vi "Initialize Generate with Scheduler.vi"(8 "error in (no error)":errorcluster, 10 "PCL (usec)":u32, 11 "OnCompile Variables":T1={"Name"="", "XNET Settings"={"Database"="", "Cluster"="", "Port"="", "Baud rate [Bd]"=500000, "Termination"=1, "CAN I/O Mode"=0, "FD Baud rate [Bd]"=500000, "Priority"=100, "Use Legacy"=FALSE, "FD ISO Mode"=0, "Default Max Counter Value"=0.0, "Default Protect Type"=enum."Arb ID + Bytes Checksum with Inversion", "Include All Channels"=FALSE}, "Frames"=[], "986x Support"={"Enable"=FALSE, "RIO Device"="", "Bitfile"=path ""}, "Incoming Frames"=[]} {"Incoming Frames"."Protection Configurations"."CRC Channels"."Data Type" items=["Signed", "Unsigned", "IEEE Float"]; "XNET Settings"."FD ISO Mode" items=["ISO", "Non ISO", "ISO Legacy"]; "XNET Settings"."CAN I/O Mode" items=["CAN 2.0", "CAN FD", "CAN FD+BRS"]; "XNET Settings"."Termination" items=["Off", "On"]; "Frames"."Protection Configurations"."CRC Channels"."Data Type" items=["Signed", "Unsigned", "IEEE Float"]}) -> (0 "error out":errorcluster, 2 "RT Configuration":T11={"Name"="", "Priority"=100, "XNET Settings"={"Database"="", "Cluster"="", "Port"="", "Baud rate [Bd]"=0, "Termination"=0, "CAN I/O Mode"=0, "FD Baud rate [Bd]"=500000, "Priority"=100, "Use Legacy"=FALSE, "FD ISO Mode"=0, "Default Max Counter Value"=0.0, "Default Protect Type"=enum."Arb ID + Bytes Checksum with Inversion", "Include All Channels"=FALSE}, "FPGA Session"=0, "Outgoing CAN Session"="", "Outgoing Cyclic Frame Count"=0, "Outgoing Cyclic Frames"=[], "Outgoing Event Frame Count"=0, "Outgoing Event Frames"=[], "Incoming CAN Session"="", "Incoming Frame Count"=0, "Incoming Frames"=[], "Incoming Values"={"Signal Values"=[], "Signal Invalid Values"=[], "ProtCtr Sig Values"=[], "Timestamps"=[], "Time Differences"=[], "IDs"=[]}} {"Outgoing Event Frames"."Protection Configurations"."CRC Channels"."Data Type" items=["Signed", "Unsigned", "IEEE Float"]; "Incoming Frames"."Protection Configurations"."CRC Channels"."Data Type" items=["Signed", "Unsigned", "IEEE Float"]; "XNET Settings"."FD ISO Mode" items=["ISO", "Non ISO", "ISO Legacy"]; "XNET Settings"."CAN I/O Mode" items=["CAN 2.0", "CAN FD", "CAN FD+BRS"]; "XNET Settings"."Termination" items=["Off", "On"]; "Outgoing Cyclic Frames"."Protection Configurations"."CRC Channels"."Data Type" items=["Signed", "Unsigned", "IEEE Float"]}, 3 "OnCompile Variables out":T1={"Name"="", "XNET Settings"={"Database"="", "Cluster"="", "Port"="", "Baud rate [Bd]"=500000, "Termination"=1, "CAN I/O Mode"=0, "FD Baud rate [Bd]"=500000, "Priority"=100, "Use Legacy"=FALSE, "FD ISO Mode"=0, "Default Max Counter Value"=0.0, "Default Protect Type"=enum."Arb ID + Bytes Checksum with Inversion", "Include All Channels"=FALSE}, "Frames"=[], "986x Support"={"Enable"=FALSE, "RIO Device"="", "Bitfile"=path ""}, "Incoming Frames"=[]} {"Incoming Frames"."Protection Configurations"."CRC Channels"."Data Type" items=["Signed", "Unsigned", "IEEE Float"]; "XNET Settings"."FD ISO Mode" items=["ISO", "Non ISO", "ISO Legacy"]; "XNET Settings"."CAN I/O Mode" items=["CAN 2.0", "CAN FD", "CAN FD+BRS"]; "XNET Settings"."Termination" items=["Off", "On"]; "Frames"."Protection Configurations"."CRC Channels"."Data Type" items=["Signed", "Unsigned", "IEEE Float"]})   [LabVIEW 2026]
uses:
  Addon Shared/Types/Exported.OnCompile.ctl
  Addon Shared/Types/XNET Settings.ctl
  SubModules/Frame-Protection-Support/Source/Shared/Types/Protection Type.ctl
  SubModules/Frame-Protection-Support/Source/Shared/Types/Exported Frame Settings.ctl
  SubModules/Frame-Protection-Support/Source/Shared/Types/Exported Frame Type.ctl
  SubModules/Frame-Protection-Support/Source/Shared/Types/Exported Protection Settings.ctl
  SubModules/Frame-Protection-Support/Source/Shared/Types/XNET Signal Configuration.ctl
  SubModules/Frame-Protection-Support/Source/Shared/Types/Exported Counter Settings.ctl
  SubModules/Frame-Protection-Support/Source/Shared/Types/Exported Event Trigger Type.ctl
  Addon Shared/Types/986x.ctl
  Types/RT Async Engine Settings.ctl
  SubModules/Frame-Protection-Support/Source/Engine/Types/RT Frame Settings.ctl
  SubModules/Frame-Protection-Support/Source/Engine/Types/RT Protection Configuration.ctl
  SubModules/Frame-Protection-Support/Source/Engine/Types/RT Frame Incoming Values.ctl
  Bitfile.Download.vi
  <vilib>/Utility/libraryn.llb/Check if File or Folder Exists.vi
  <vilib>/Utility/error.llb/Error Cluster From Error Code.vi
  <vilib>/rvi/Utilities/XML/nirviXML_GetValue.vi
  <vilib>/rvi/Utilities/XML/nirviXML_GetValue_String.vi
  <vilib>/xnet/xnet.llb/XNET Create Session (Frame Output Stream).vi
  <vilib>/xnet/xnet.llb/XNET Create Session (Conversion).vi
  SubModules/Frame-Protection-Support/Source/Shared/Protection and Counter Support Shared.lvlib
  SubModules/Frame-Protection-Support/Source/Engine/Protection and Counter Support Engine.lvlib
  Protection and Counter Addon Engine.lvlib
  <resource>/objmgr/xnet.rc
  Addon Shared/Protection and Counter Addon Shared.lvlib
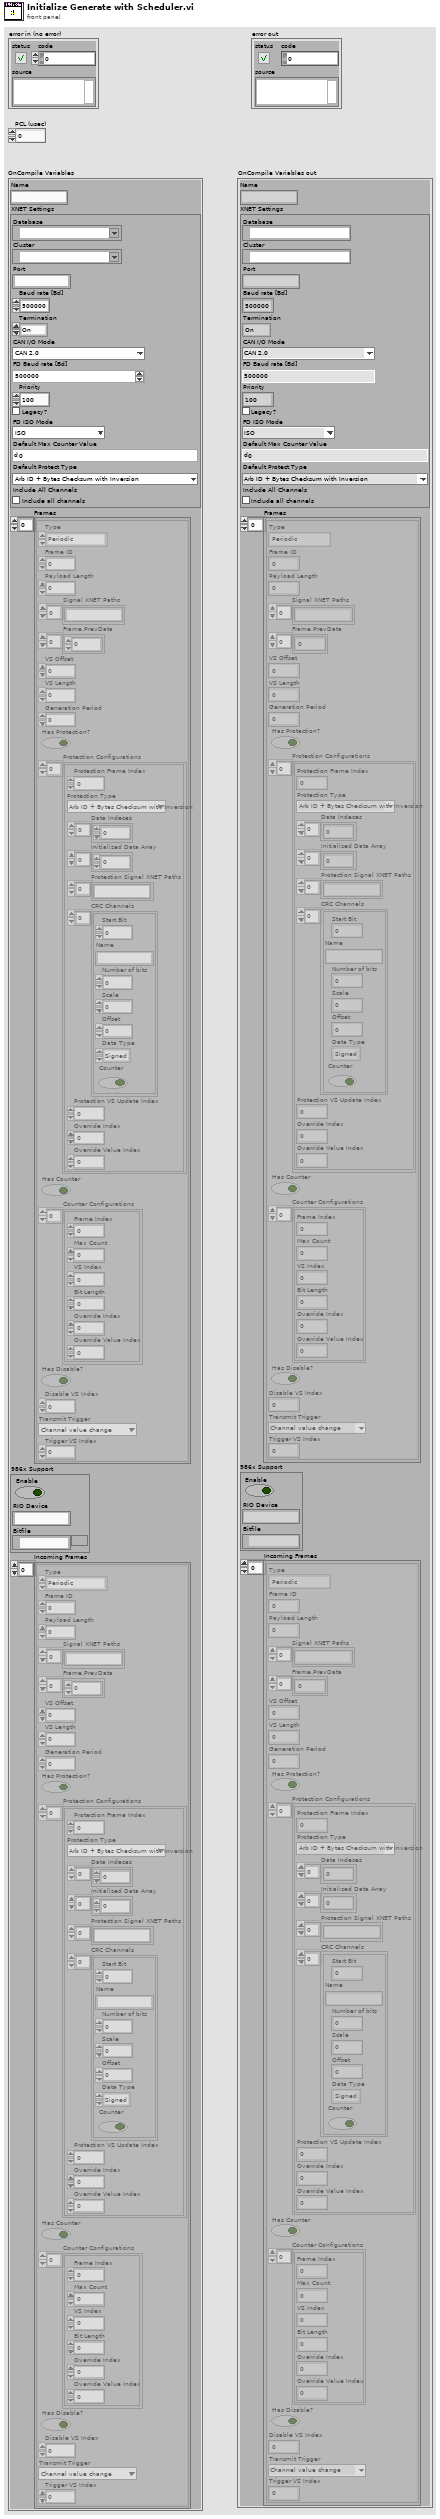
[diagram p1: front panel]
types:
  T1 = typedef "Protection and Counter Addon Shared.lvlib/Exported.OnCompile.ctl" = cluster{"Name":string, "XNET Settings":T2, "Frames":T4[], "986x Support":T10, "Incoming Frames":T4[]}
  T2 = typedef "Protection and Counter Addon Shared.lvlib/XNET Settings.ctl" = cluster{"Database":refnum<k21>, "Cluster":refnum<k21>, "Port":string, "Baud rate [Bd]":u64, "Termination":u32, "CAN I/O Mode":u32, "FD Baud rate [Bd]":u64, "Priority":i32, "Use Legacy":bool, "FD ISO Mode":u32, "Default Max Counter Value":dbl, "Default Protect Type":T3, "Include All Channels":bool}
  T3 = typedef "Protection and Counter Support Shared.lvlib/Protection Type.ctl" = enum16{"Arb ID + Bytes Checksum with Inversion", "Arb ID + Bytes CRC with Inversion", "Reversed Raw Signal Checksum with Inversion", "Concatenated Two's Compliment"}
  T4 = typedef "Protection and Counter Support Shared.lvlib/Exported Frame Settings.ctl" = cluster{"Type":T5, "Frame ID":u32, "Payload Length":u32, "Signal XNET Paths":string[], "Frame.PrevData":dbl[], "VS Offset":i32, "VS Length":i32, "Generation Period":u32, "Has Protection?":bool, "Protection Configurations":T6[], "Has Counter":bool, "Counter Configurations":T8[], "Has Disable?":bool, "Disable VS Index":i32, "Transmit Trigger":T9, "Trigger VS Index":i32}
  T5 = typedef "Protection and Counter Support Shared.lvlib/Exported Frame Type.ctl" = enum16{"Periodic", "Event", "Periodic/Event"}
  T6 = typedef "Protection and Counter Support Shared.lvlib/Exported Protection Settings.ctl" = cluster{"Protection Frame Index":i32, "Protection Type":T3, "Data Indeces":i32[], "Initialized Data Array":dbl[], "Protection Signal XNET Paths":string[], "CRC Channels":T7[], "Protection VS Update Index":i32, "Override Index":i32, "Override Value Index":i32}
  T7 = typedef "Protection and Counter Support Shared.lvlib/XNET Signal Configuration.ctl" = cluster{"Start Bit":i32, "Name":string, "Number of bits":i32, "Scale":dbl, "Offset":dbl, "Data Type":u32, "Counter":bool}
  T8 = typedef "Protection and Counter Support Shared.lvlib/Exported Counter Settings.ctl" = cluster{"Frame Index":i32, "Max Count":dbl, "VS Index":i32, "Bit Length":i64, "Override Index":i32, "Override Value Index":i32}
  T9 = typedef "Protection and Counter Support Shared.lvlib/Exported Event Trigger Type.ctl" = enum16{"Channel value change", "Trigger channel (not zero)", "Channel value change or trigger channel (not zero)", "Trigger channel (any value change)", "Channel value change or trigger channel (any value change)"}
  T10 = typedef "Protection and Counter Addon Shared.lvlib/986x.ctl" = cluster{"Enable":bool, "RIO Device":string, "Bitfile":path}
  T11 = typedef "Protection and Counter Addon Engine.lvlib/RT Async Engine Settings.ctl" = cluster{"Name":string, "Priority":i32, "XNET Settings":T2, "FPGA Session":u32, "Outgoing CAN Session":refnum<k21>, "Outgoing Cyclic Frame Count":i32, "Outgoing Cyclic Frames":T12[], "Outgoing Event Frame Count":i32, "Outgoing Event Frames":T12[], "Incoming CAN Session":refnum<k21>, "Incoming Frame Count":i32, "Incoming Frames":T12[], "Incoming Values":T14}
  T12 = typedef "Protection and Counter Support Engine.lvlib/RT Frame Settings.ctl" = cluster{"Type":T5, "Frame ID":u32, "Payload Length":u32, "VS Offset":i32, "VS Length":i32, "Frame Conversion":refnum<k21>, "Frame.Data":dbl[], "Generation Period":u32, "Time Since Last Generation":u32, "Generation Iterations":u32, "Generation Counter":u32, "Has Protection?":bool, "Protection Configurations":T13[], "Has Counter?":bool, "Counter Configurations":T8[], "Has Disable?":bool, "Disable VS Index":i32, "Transmit Trigger":T9, "Trigger VS Index":i32}
  T13 = typedef "Protection and Counter Support Engine.lvlib/RT Protection Configuration.ctl" = cluster{"Protection Frame Index":i32, "Protection Type":T3, "Data Indeces":i32[], "Data Array":dbl[], "Check Sum Conversion":refnum<k21>, "CRC Channels":T7[], "Protection VS Index":i32, "Counter Data Index":i32, "Override Index":i32, "Override Value Index":i32}
  T14 = typedef "Protection and Counter Support Engine.lvlib/RT Frame Incoming Values.ctl" = cluster{"Signal Values":dbl[], "Signal Invalid Values":dbl[], "ProtCtr Sig Values":dbl[], "Timestamps":timestamp[], "Time Differences":dbl[], "IDs":u32[]}
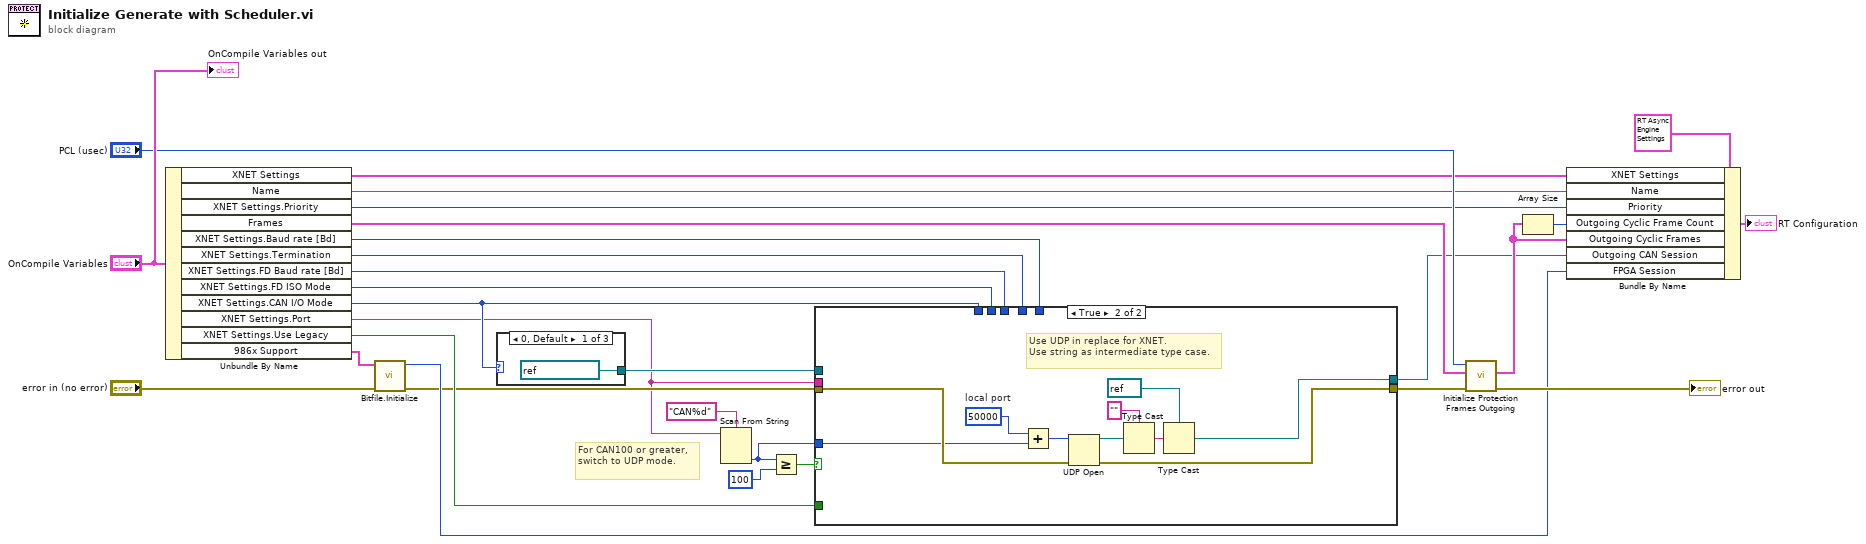
[diagram p0: block diagram]
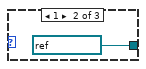
[diagram p2: hidden frame]
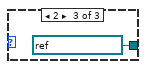
[diagram p3: hidden frame]
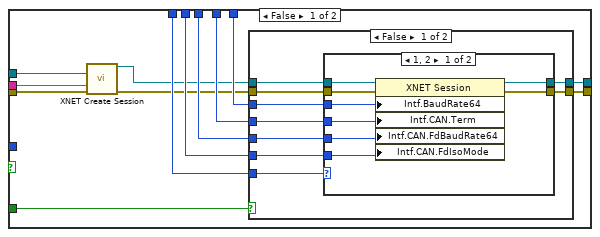
[diagram p4: hidden frame]
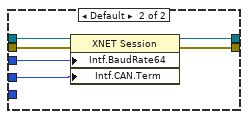
[diagram p5: hidden frame]
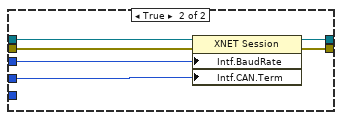
[diagram p6: hidden frame]
diagram:
  # "For CAN100 or greater, switch to UDP mode."
  n1 = Unbundle By Name("OnCompile Variables") -> ("XNET Settings"=w11:T2, "Name"=w12:string, "XNET Settings.Priority"=w18:i32, "Frames"=w28:T4[], "XNET Settings.Baud rate [Bd]"=w21:u64, "XNET Settings.Termination"=w22:u32, "XNET Settings.FD Baud rate [Bd]"=w23:u64, "XNET Settings.FD ISO Mode"=w9:u32, "XNET Settings.CAN I/O Mode"=w8:u32, "XNET Settings.Port"=w4:string, "XNET Settings.Use Legacy"=w17:bool, "986x Support"=w16:T10)
  n2 = call "Bitfile.Initialize.vi"("error in (no error)"="error in (no error)", "FPGA Bitfile Settings"=w16) -> ("error out"=w6:errorcluster, "FPGA Session"=w15:u32)  [unwired: 8 in]
  n3 = case shown="0, Default" w8 {
    tunnel: [refnum<k21> ":memory:" ("cluster (:memory:)") refnum<k21> ":can_fd:" ("cluster (:memory:)") refnum<k21> ":can_fd_brs:" ("cluster (:memory:)")] -> w10
    frame 0, Default {
    }
    frame 1 {
    }
    frame 2 {
    }
  }
  n4 = Scan From String(format string="CAN%d", input string=w4) -> (output 1=w1:i32)  [unwired: 3 in, 3 out]
  n5 = Greater Or Equal?(x=w1, y=100) -> (x >= y?=w2:bool)
  n6 = case shown="True" w2 {
    tunnel: [w45 w78] -> w24
    tunnel: w23 -> [w44 _]
    tunnel: w22 -> [w43 _]
    tunnel: w21 -> [w42 _]
    tunnel: w17 -> [w41 _]
    tunnel: [w40 w79] -> w13
    tunnel: w10 -> [w39 _]
    tunnel: w9 -> [w38 _]
    tunnel: w8 -> [w37 _]
    tunnel: w6 -> [w36 w80]
    tunnel: w4 -> [w35 _]
    tunnel: w1 -> [_ w76]
    frame False {
      n7 = call-poly <vilib>:"XNET Create Session.vi"("cluster (:memory:)"=w39, "interface"=w35, "error in (no error)"=w36) -> ("session out"=w34:refnum<k21>, "error out"=w33:errorcluster)  [unwired: 11 in]
      n8 = case shown="False" w41 {
        tunnel: w33 -> [w54 w74]
        tunnel: w34 -> [w53 w73]
        tunnel: [w52 w72] -> w45
        tunnel: w44 -> [w51 _]
        tunnel: w37 -> [w47 _]
        tunnel: w43 -> [w50 w69]
        tunnel: w42 -> [w49 w70]
        tunnel: [w48 w71] -> w40
        tunnel: w38 -> [w46 _]
        frame False {
          n9 = case shown="1, 2" w47 {
            tunnel: w54 -> [w62 w68]
            tunnel: w53 -> [w61 w67]
            tunnel: [w60 w66] -> w52
            tunnel: w51 -> [w59 _]
            tunnel: w50 -> [w58 w65]
            tunnel: w49 -> [w57 w64]
            tunnel: [w56 w63] -> w48
            tunnel: w46 -> [w55 _]
            frame 1, 2 {
              n10 = property class="XNET Session"(reference=w61, error in=w62, "Intf.BaudRate64"=w57, "Intf.CAN.Term"=w58, "Intf.CAN.FdBaudRate64"=w59, "Intf.CAN.FdIsoMode"=w55) -> (reference out=w56:refnum<k21>, error out=w60:errorcluster)
            }
            frame Default {
              n11 = property class="XNET Session"(reference=w67, error in=w68, "Intf.BaudRate64"=w64, "Intf.CAN.Term"=w65) -> (reference out=w63:refnum<k21>, error out=w66:errorcluster)
            }
          }
        }
        frame True {
          n12 = property class="XNET Session"(reference=w73, error in=w74, "Intf.BaudRate"=w70, "Intf.CAN.Term"=w69) -> (reference out=w71:refnum<k21>, error out=w72:errorcluster)
        }
      }
    }
    frame True {
      w77 = u16 50000  # local port
      # "Use UDP in replace for XNET.\nUse string as intermediate type case."
      n13 = Add(x=w77, y=w76) -> (x+y=w75:i32)
      n14 = UDP Open(8:w80, 11:w75) -> (port=w83:refnum<k16>, 0:w78:errorcluster)  [unwired: 3 in, 1 out]
      n15 = Type Cast(type="", x=w83) -> (*(type *) &x=w84:string)
      n16 = Type Cast(type=refnum<k21> refnum ("session out"), x=w84) -> (*(type *) &x=w79:refnum<k21>)
    }
  }
  n17 = call "Initialize Protection Frames Outgoing.vi"("error in (no error)"=w24, "Frames"=w28, "PCL (usec)"="PCL (usec)") -> ("error out"=→"error out":errorcluster, "RT Frames"=w14:T12[])  [unwired: 7 in]
  n18 = Array Size(array=w14) -> (size(s)=w19:i32)
  n19 = Bundle By Name(cluster=T11 {"Name"="", "Priority"=100, "XNET Settings"={"Database"="", "Cluster"="", "Port"="", "Baud rate [Bd]"=0, "Termination"=0, "CAN I/O Mode"=0, "FD Baud rate [Bd]"=500000, "Priority"=100, "Use Legacy"=FALSE, "FD ISO Mode"=0, "Default Max Counter Value"=0.0, "Default Protect Type"=enum."Arb ID + Bytes Checksum with Inversion", "Include All Channels"=FALSE}, "FPGA Session"=0, "Outgoing CAN Session"="", "Outgoing Cyclic Frame Count"=0, "Outgoing Cyclic Frames"=[], "Outgoing Event Frame Count"=0, "Outgoing Event Frames"=[], "Incoming CAN Session"="", "Incoming Frame Count"=0, "Incoming Frames"=[], "Incoming Values"={"Signal Values"=[], "Signal Invalid Values"=[], "ProtCtr Sig Values"=[], "Timestamps"=[], "Time Differences"=[], "IDs"=[]}} ("RT Configuration"), "XNET Settings"=w11, "Name"=w12, "Priority"=w18, "Outgoing Cyclic Frame Count"=w19, "Outgoing Cyclic Frames"=w14, "Outgoing CAN Session"=w13, "FPGA Session"=w15) -> (→"RT Configuration":T11)
  "OnCompile Variables out" <- "OnCompile Variables"
